vi "Create directory.vi"(8 "error in (no error)":errorcluster, 10 "Directory":string, 11 "SCP File Transfer in":refnum<class "SCP File Transfer.lvclass">) -> (0 "error out":errorcluster, 3 "SCP File Transfer out":refnum<class "SCP File Transfer.lvclass">)   [LabVIEW 2014, in "PL Framework Configuration Tool.lvlib" / "SCP File Transfer.lvclass"]
doc: "Creates the \"Directory\" on the remote target. The VI also creates all needed directories if the \"Directory\" path contains directories that don't exist on the target.\n\nThe recommended file path format for \"Remote path\" is \"/directory1/directory2\". However, the VI will accept other formats and transform the path appropriately in most cases. Use the \"Strip path.vi\" and \"Build path.vi\" VIs to help with handling remote path strings."
uses:
  SCP File Transfer.lvclass
  SCP File Transfer.lvclass/SCP File Transfer.ctl
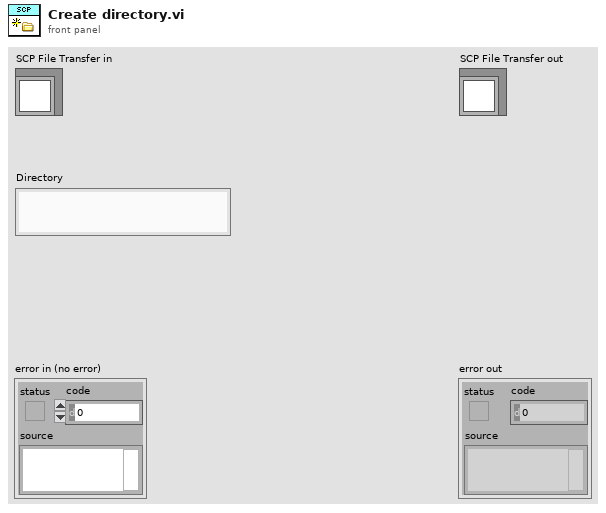
[diagram p1: front panel]
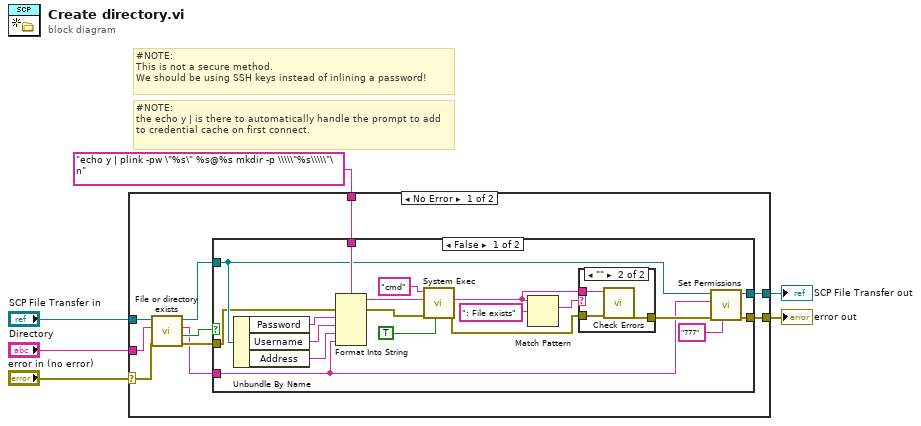
[diagram p0: block diagram]
diagram:
  # "#NOTE:\nthe echo y | is there to automatically handle the prompt to add to credential cache on first connect."
  # "#NOTE:\nThis is not a secure method.\nWe should be using SSH keys instead of inlining a password!"
  n1 = case shown="No Error" "error in (no error)" {
    selector: "error in (no error)" -> [w10 w42]
    tunnel: "echo y | plink -pw \"%s\" %s@%s mkdir -p \\\\\"%s\\\\\"\n" ("format string") -> [w16 _]
    tunnel: "Directory" -> [w11 _]
    tunnel: "SCP File Transfer in" -> [w13 w43]
    tunnel: [w15 w43] -> w3
    tunnel: [w14 w42] -> w2
    frame No Error {
      n2 = call-dynamic "File or directory exists.vi"("error in (no error)"=w10, "Path"=w11, "SCP File Transfer in"=w13) -> ("error out"=w9:errorcluster, "Exists?"=w8:bool, "Path out (dup)"=w7:string, "SCP File Transfer out"=w12:refnum<class "SCP File Transfer.lvclass">)  [unwired: 4 in, 1 out]
      n3 = case shown="False" w8 {
        tunnel: w16 -> [w34 _]
        tunnel: w7 -> [w27 _]
        tunnel: w12 -> [w26 w41]
        tunnel: [w23 w41] -> w15
        tunnel: [w22 w40] -> w14
        tunnel: w9 -> [w18 w40]
        frame False {
          n4 = Unbundle By Name(w26) -> ("Password"=w25:string, "Username"=w30:string, "Address"=w24:string)
          n5 = Format Into String(format string=w34, error in=w18, w25, w30, w24, w27) -> (resulting string=w31:string, error out=w35:errorcluster)  [unwired: 1 in]
          n6 = call <vilib>:"System Exec.vi"("run minimized? (F)"=TRUE, "error in (no error)"=w35, "standard input"=w31, "command line"="cmd") -> ("error out"=w32:errorcluster, "standard error"=w19:string)  [unwired: 4 in, 2 out]
          n7 = Match Pattern(string=w19, regular expression=": File exists") -> (match substring=w20:string)  [unwired: 1 in, 3 out]
          n8 = case shown="\"\"" w20 {
            tunnel: w32 -> [w36 w39]
            tunnel: [w36 w38] -> w28
            tunnel: w19 -> [_ w37]
            frame Default {
            }
            frame "" {
              n9 = call "Check Errors.vi"("error in (no error)"=w39, "standard error"=w37) -> ("error out"=w38:errorcluster)  [unwired: 9 in]
            }
          }
          n10 = call "Set Permissions.vi"("permissions"="777", "error in (no error)"=w28, "Remote path"=w27, "SCP File Transfer in"=w26) -> ("error out"=w22:errorcluster, "SCP File Transfer out"=w23:refnum<class "SCP File Transfer.lvclass">)  [unwired: 6 in]
        }
        frame True {
        }
      }
    }
    frame Error {
    }
  }
  "error out" <- w2
  "SCP File Transfer out" <- w3
